vi "_Raise Navigation Starting Event.vi"(4 "WebView2.lvlib:WebView2 Control.lvclass":refnum<class "WebView2 Control.lvclass">, 5 "Event Data":cluster{"sender":refnum<k24>, "e":refnum<k24>}, 6 "Control Ref":refnum<k24>, 7 "Event Common Data":T1) -> ()   [LabVIEW 2020, in "WebView2.lvlib" / "WebView2 Control.lvclass"]
uses:
  WebView2 Control.lvclass
  E:/Labview/LV 2023/PPL/PPL Builder/Libs/LV-WebView2/Source/Libs/Microsoft.Web.WebView2.Core.dll
  Libs/Microsoft.Web.WebView2.Core.dll
  WebView2 Event Filter Interface/WebView2 Event Filter Interface.lvclass
  WebView2 Control.lvclass/WebView2 Control.ctl
  Navigation Start Event Data.ctl
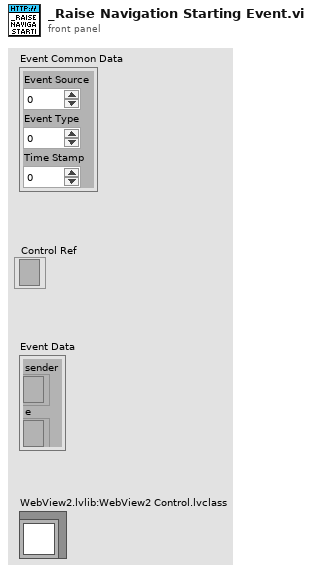
[diagram p1: front panel]
types:
  T1 = cluster{"Event Source":i32, "Event Type":u32, "Time Stamp":u32}
  T2 = typedef "WebView2.lvlib/WebView2 Control.lvclass/Navigation Start Event Data.ctl" = cluster{"AdditionalAllowedFrameAncestors":string, "IsRedirected":bool, "IsUserInitiated":bool, "NavigationId":u64, "NavigationKind":i32, "Uri":string, "Headers":cluster{"Key":string, "Value":string}[], "Event Filter":refnum<class "WebView2 Event Filter Interface.lvclass">}
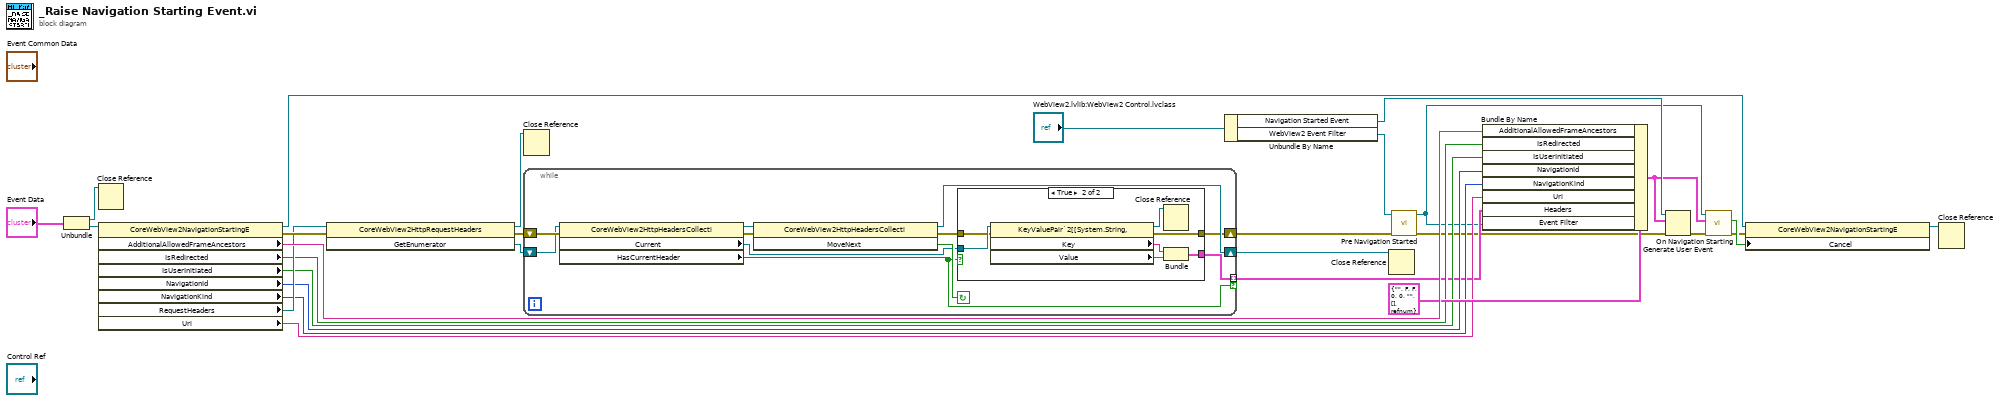
[diagram p0: block diagram]
diagram:
  n1 = Unbundle("Event Data") -> ("sender"=w24:refnum<k24>, "e"=w17:refnum<k24>)
  n2 = Close Reference(reference=w24) -> ()  [unwired: 1 in, 1 out]
  n3 = property class="CoreWebView2NavigationStartingE"(reference=w17) -> (reference out=w16:refnum<k24>, error out=w20:errorcluster, "AdditionalAllowedFrameAncestors"=w26:string, "IsRedirected"=w15:bool, "IsUserInitiated"=w14:bool, "NavigationId"=w13:u64, "NavigationKind"=w12:i32, "RequestHeaders"=w18:refnum<k24>, "Uri"=w11:string)  [unwired: 1 in]
  n4 = invoke class="CoreWebView2HttpRequestHeaders" method="GetEnumerator"(reference=w18, error in=w20) -> (reference out=w19:refnum<k24>, error out=w22:errorcluster, "GetEnumerator"=w23:refnum<k24>)  [unwired: 1 in]
  n5 = Close Reference(reference=w19) -> ()  [unwired: 1 in, 1 out]
  n6 = while {
    shift-right: [w33] -> w21
    shift-left: w23 -> [w37]
    shift-right: [w31] -> w2
    shift-left: w22 -> [w39]
    tunnel: [w34] -> w10 mode=indexing if=w30
    stop <- w40 continue-if-true
    n7 = property class="CoreWebView2HttpHeadersCollecti"(reference=w37, error in=w39) -> (reference out=w36:refnum<k24>, error out=w38:errorcluster, "Current"=w35:refnum<k24>, "HasCurrentHeader"=w30:bool)
    n8 = invoke class="CoreWebView2HttpHeadersCollecti" method="MoveNext"(reference=w36, error in=w38) -> (reference out=w33:refnum<k24>, error out=w32:errorcluster, "MoveNext"=w40:bool)  [unwired: 1 in]
    n9 = case shown="True" w30 {
      tunnel: w35 -> [_ w48]
      tunnel: [_ w45] -> w34
      tunnel: w32 -> [w41 w43]
      tunnel: [w41 w42] -> w31
      frame False {
      }
      frame True {
        n10 = property class="KeyValuePair`2[[System.String, "(reference=w48, error in=w43) -> (reference out=w44:refnum<k24>, error out=w42:errorcluster, "Key"=w47:string, "Value"=w46:string)
        n11 = Close Reference(reference=w44) -> ()  [unwired: 1 in, 1 out]
        n12 = Bundle("Key"=w47, "Value"=w46) -> (w45:cluster{"Key":string, "Value":string})  [unwired: 1 in]
      }
    }
  }
  n13 = Unbundle By Name("WebView2.lvlib:WebView2 Control.lvclass") -> ("Navigation Started Event"=w29:refnum<user-event>, "WebView2 Event Filter"=w8:refnum<class "WebView2 Event Filter Interface.lvclass">)
  n14 = Close Reference(reference=w21) -> ()  [unwired: 1 in, 1 out]
  n15 = call-dynamic "Pre Navigation Started.vi"("error in (no error)"=w2, "WebView2 Event Filter Interface in"=w8) -> ("error out"=w1:errorcluster, "WebView2 Event Filter Interface out"=w7:refnum<class "WebView2 Event Filter Interface.lvclass">)  [unwired: 8 in]
  n16 = Bundle By Name(cluster=T2 {"AdditionalAllowedFrameAncestors"="", "IsRedirected"=FALSE, "IsUserInitiated"=FALSE, "NavigationId"=0, "NavigationKind"=0, "Uri"="", "Headers"=[], "Event Filter"=refnum} ("Nav Started Event"), "AdditionalAllowedFrameAncestors"=w26, "IsRedirected"=w15, "IsUserInitiated"=w14, "NavigationId"=w13, "NavigationKind"=w12, "Uri"=w11, "Headers"=w10, "Event Filter"=w7) -> (w6:T2)
  n17 = Generate User Event(user event=w29, event data cluster=w6, error in=w1) -> (error out=w4:errorcluster)  [unwired: 1 in, 1 out]
  n18 = call-dynamic "On Navigation Starting.vi"("error in (no error)"=w4, "Nav Started Event"=w6, "WebView2 Event Filter Interface in"=w7) -> ("error out"=w3:errorcluster, "Cancel"=w5:bool)  [unwired: 7 in]
  n19 = property class="CoreWebView2NavigationStartingE"(reference=w16, error in=w3, "Cancel"=w5) -> (reference out=w9:refnum<k24>)  [unwired: 1 out]
  n20 = Close Reference(reference=w9) -> ()  [unwired: 1 in, 1 out]
